vi "Main.vi"(8 "error in":errorcluster, 10 "User Events":T1, 11 "Message Queues in":T2) -> (0 "error out":errorcluster)   [LabVIEW 2026, in "UI.lvlib"]
doc: "This template is for the Queued Message Handler design pattern.\n\nThe Event Handling Loop generates messages based on user interface actions.\n\nThe Message Handling Loop processes messages generated by the Event Handling Loop, or by other messages. The messages are string values, so new messages can be added easily to the Message Cases case structure in the Message Handling Loop. Each message cluster can also provide an optional value for Message Data, which is a variant that can be converted to whatever message-specific data is required."
uses:
  UI.lvlib
  support/Message Queue/All Message Queues.ctl
  support/Message Queue/Message Cluster.ctl
  support/User Event - Stop/User Events.ctl
  Type Definitions/Data.ctl
  63137d18-bf8a-4e88-9200-6af118f85cfe.vi
  1e39ca58-9476-46a2-b025-c1705f3df17d.vi
  996e5f3e-9492-4e2b-97a9-5cb558c20b1f.vi
  73755cc0-1500-4328-8249-424498ba1049.vi
  5d810f25-301b-4729-8d99-398627275c85.vi
  4f3ed8a2-4889-49b4-8636-eb87dbb66537.vi
  c1dd759d-c855-4646-8354-c3344e12efab.vi
  4da0cbbb-3ae4-43c8-84ea-24bb95110d96.vi
  72e6443c-2ce6-4ed8-b611-5763f8d8c9de.vi
  63137d18-bf8a-4e88-9200-6af118f85cfe.vi/904feb24-0ee5-4d46-a973-81b984403c80.vi
  1e39ca58-9476-46a2-b025-c1705f3df17d.vi/904feb24-0ee5-4d46-a973-81b984403c80.vi
  996e5f3e-9492-4e2b-97a9-5cb558c20b1f.vi/904feb24-0ee5-4d46-a973-81b984403c80.vi
  73755cc0-1500-4328-8249-424498ba1049.vi/904feb24-0ee5-4d46-a973-81b984403c80.vi
  5d810f25-301b-4729-8d99-398627275c85.vi/904feb24-0ee5-4d46-a973-81b984403c80.vi
  4f3ed8a2-4889-49b4-8636-eb87dbb66537.vi/904feb24-0ee5-4d46-a973-81b984403c80.vi
  c1dd759d-c855-4646-8354-c3344e12efab.vi/904feb24-0ee5-4d46-a973-81b984403c80.vi
  4da0cbbb-3ae4-43c8-84ea-24bb95110d96.vi/904feb24-0ee5-4d46-a973-81b984403c80.vi
  72e6443c-2ce6-4ed8-b611-5763f8d8c9de.vi/904feb24-0ee5-4d46-a973-81b984403c80.vi
  support/Message Queue/Enqueue Message (Single).vi
  <vilib>/Utility/error.llb/Error Cluster From Error Code.vi
  <vilib>/ErrorRing/Error Ring.xnode
  support/Message Queue/Message Queue.lvlib
  support/User Event - Stop/User Event - Stop.lvlib
panel:
  out "Display <Replace Me>":string
  in  "Do Something Else <Replace Me>":bool
  in  "Do Something <Replace Me>":bool
  in  "Exit":bool
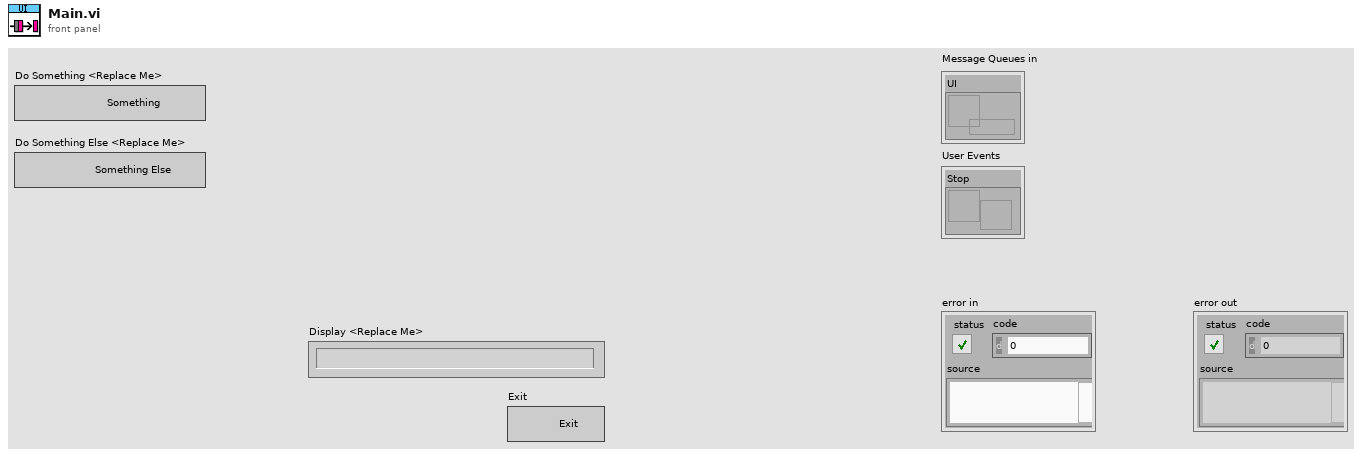
[diagram p1: front panel]
types:
  T1 = typedef "User Event - Stop.lvlib/User Events.ctl" = cluster{"Stop":refnum<user-event>}
  T2 = typedef "Message Queue.lvlib/All Message Queues.ctl" = cluster{"UI":refnum<queue>}
  T3 = enum32{"Invalid", "Standard", "Closed", "Hidden", "Minimized", "Maximized"}
  T4 = typedef "UI.lvlib/Data.ctl" = cluster{"Boolean <Replace Me>":bool, "String <Replace Me>":string, "Numeric <Replace Me>":dbl, "Do Something Ref":refnum<vi>, "Do Something Else Ref":refnum<vi>, "Exit Button Ref":refnum<vi>, "Display Ref":refnum<vi>}
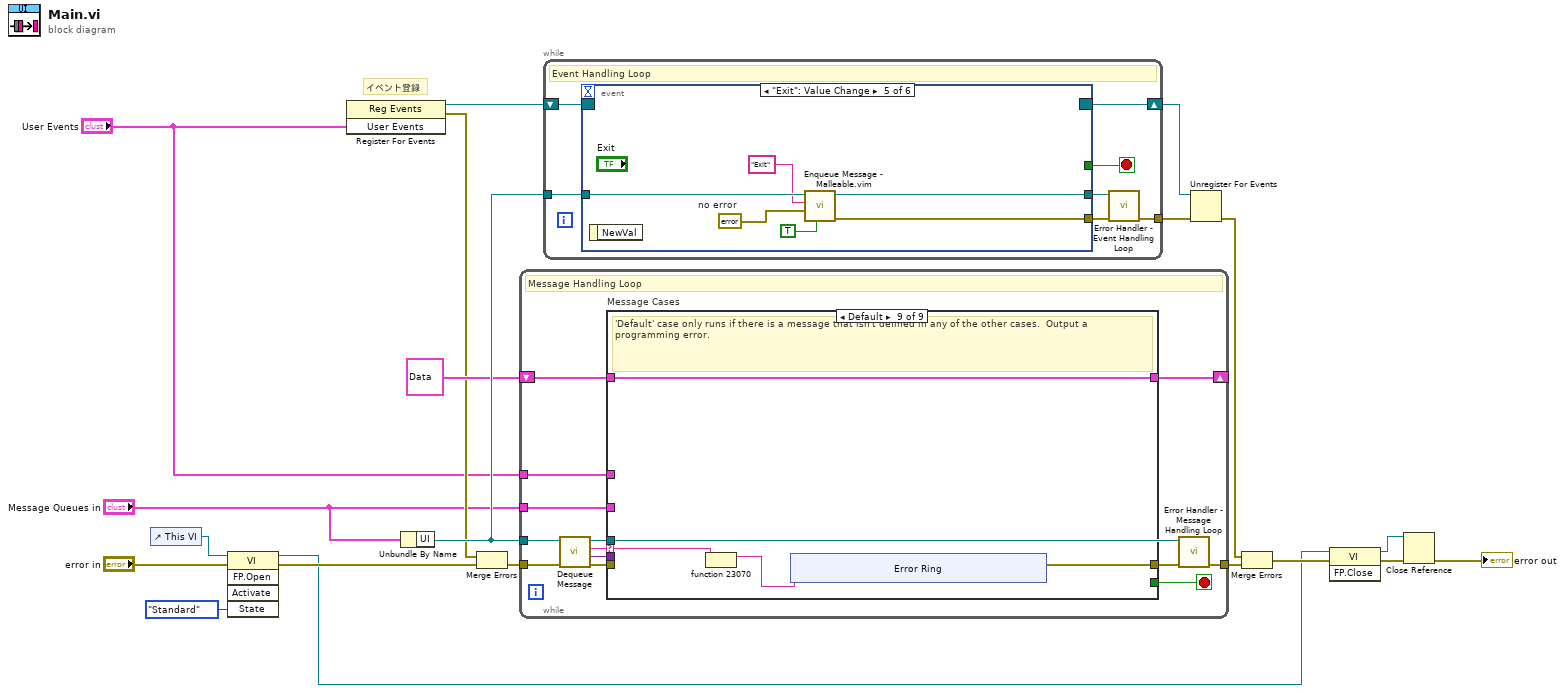
[diagram p0: block diagram]
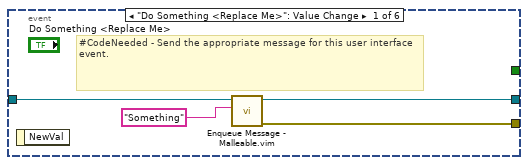
[diagram p2: hidden frame]
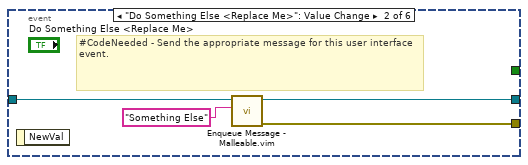
[diagram p3: hidden frame]
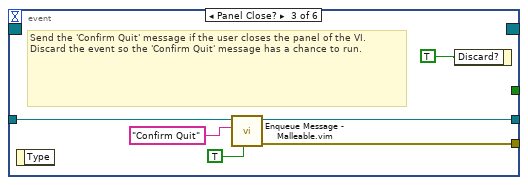
[diagram p4: hidden frame]
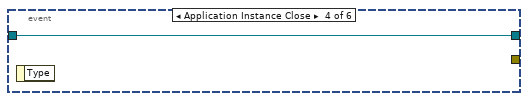
[diagram p5: hidden frame]
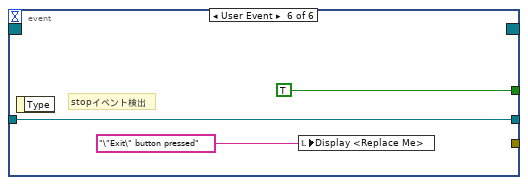
[diagram p6: hidden frame]
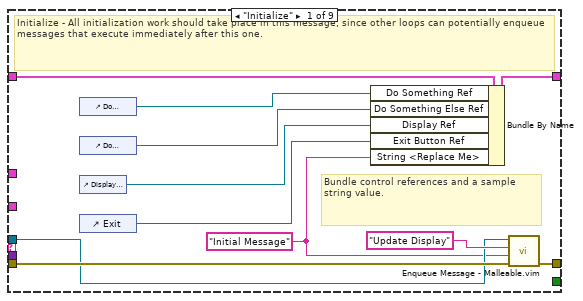
[diagram p7: hidden frame]
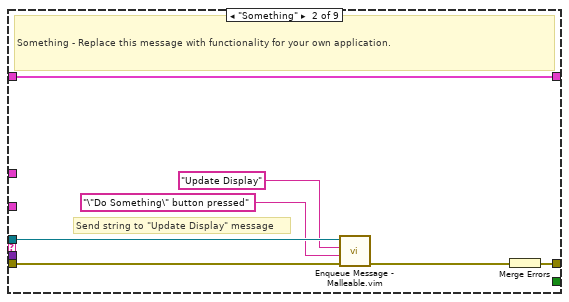
[diagram p8: hidden frame]
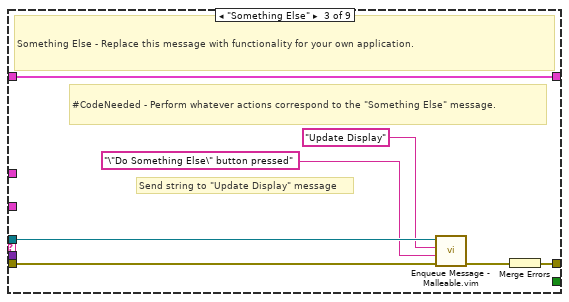
[diagram p9: hidden frame]
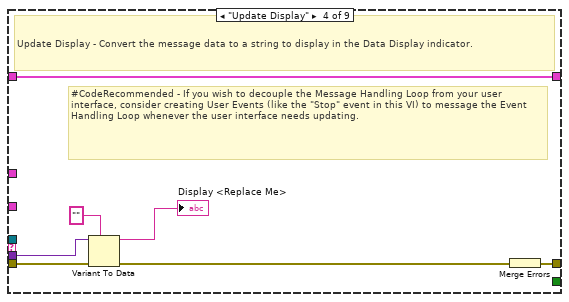
[diagram p10: hidden frame]
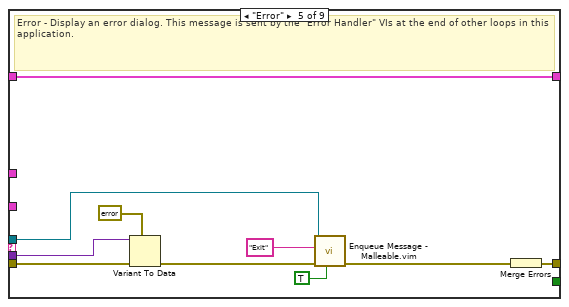
[diagram p11: hidden frame]
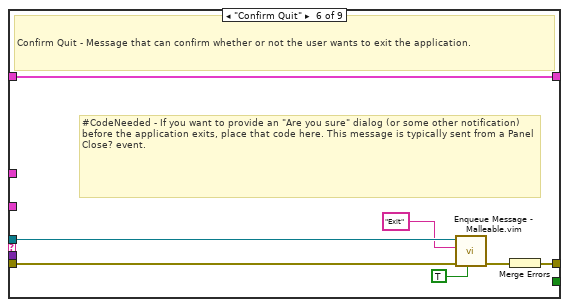
[diagram p12: hidden frame]
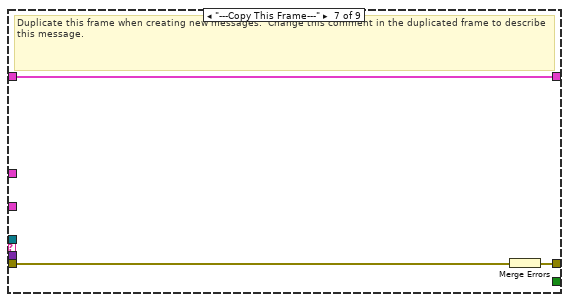
[diagram p13: hidden frame]
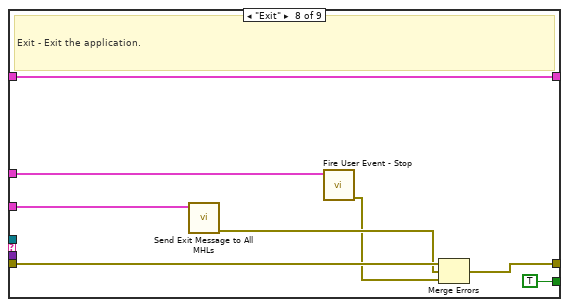
[diagram p14: hidden frame]
diagram:
  # "イベント登録"
  n1 = control-ref of="This VI"() -> (w6:refnum<vi>)
  n2 = invoke class="VI" method="FP.Open"(reference=w6, error in="error in", "State"=T3."Standard") -> (reference out=w4:refnum<vi>, error out=w7:errorcluster)  [unwired: 2 in, 3 out]
  n3 = register-events("User Events") -> (reference out=w14:refnum<event-registration>, error out=w12:errorcluster)  [unwired: 2 in]
  n4 = Unbundle By Name("Message Queues in") -> ("UI"=w19:refnum<queue>)
  n5 = Merge Errors(w12, w7) -> (w13:errorcluster)
  n6 = while {
    tunnel: w19 -> [w25]
    shift-right: [w32] -> _
    shift-left: T4 {"Boolean <Replace Me>"=FALSE, "String <Replace Me>"="", "Numeric <Replace Me>"=0.0, "Do Something Ref"=refnum, "Do Something Else Ref"=refnum, "Exit Button Ref"=refnum, "Display Ref"=refnum} ("Data Cluster") -> [w33]
    tunnel: "User Events" -> [w30]
    tunnel: w13 -> [w29]
    tunnel: [w23] -> w20
    tunnel: "Message Queues in" -> [w21]
    stop <- w31 stop-if-true
    # "Message Handling Loop"
    n7 = call "Dequeue Message.vi"("error in (no error)"=w29, "Message Queue"=w25) -> ("error out"=w28:errorcluster, "Message Data"=w26:variant, "Message"=w27:string, "dup Message Queue"=w24:refnum<queue>)  [unwired: 6 in]
    n8 = case "Message Cases" shown="Default" w27 {
      selector: w27 -> [_ _ _ _ _ _ _ _ w95]
      tunnel: w24 -> [w36 w48 w54 _ w69 w78 _ _ _]
      tunnel: w28 -> [w43 w49 w56 w63 w75 w82 w85 w88 _]
      tunnel: [w44 w50 w57 w64 w71 w80 w83 w91 w96] -> w22
      tunnel: w33 -> [w42 w51 w58 w65 w74 w81 w84 w93 w97]
      tunnel: [w41 w51 w58 w65 w74 w81 w84 w93 w97] -> w32
      tunnel: [_ _ _ _ _ _ _ TRUE _] -> w31
      tunnel: w26 -> [_ _ _ w62 w73 _ _ _ _]
      tunnel: w30 -> [_ _ _ _ _ _ _ w90 _]
      tunnel: w21 -> [_ _ _ _ _ _ _ w89 _]
      frame "Initialize" {
        w35 = "Initial Message" ("Initial Message")
        # "Bundle control references and a sample string value."
        # "Initialize - All initialization work should take place in this message, since other loops can potentially enqueue messages that execute immediately after this one."
        n9 = control-ref of="Do Something <Replace Me>"() -> (w40:refnum<vi>)
        n10 = control-ref of="Do Something Else <Replace Me>"() -> (w39:refnum<vi>)
        n11 = control-ref of="Display <Replace Me>"() -> (w34:refnum<vi>)
        n12 = control-ref of="Exit"() -> (w38:refnum<vi>)
        n13 = Bundle By Name(cluster=w42, "Do Something Ref"=w40, "Do Something Else Ref"=w39, "Display Ref"=w34, "Exit Button Ref"=w38, "String <Replace Me>"=w35) -> (w41:T4)
        n14 = call "Enqueue Message - Malleable.vim"("error in (no error)"=w43, "Message Data"=w35, "Message"="Update Display", "Message Queue"=w36) -> ("error out"=w44:errorcluster)  [unwired: 6 in, 1 out]
      }
      frame "Something" {
        # "Send string to \"Update Display\" message"
        # "Something - Replace this message with functionality for your own application."
        n15 = call "Enqueue Message - Malleable.vim"("error in (no error)"=w49, "Message Data"="\"Do Something\" button pressed" ("\"Do Something\" button pressed"), "Message"="Update Display", "Message Queue"=w48) -> ("error out"=w45:errorcluster)  [unwired: 6 in, 1 out]
        n16 = Merge Errors(w45) -> (w50:errorcluster)
      }
      frame "Something Else" {
        # "Send string to \"Update Display\" message"
        # "#CodeNeeded - Perform whatever actions correspond to the \"Something Else\" message."
        # "Something Else - Replace this message with functionality for your own application."
        n17 = call "Enqueue Message - Malleable.vim"("error in (no error)"=w56, "Message Data"="\"Do Something Else\" button pressed" ("\"Do Something Else\" button pressed"), "Message"="Update Display", "Message Queue"=w54) -> ("error out"=w55:errorcluster)  [unwired: 6 in, 1 out]
        n18 = Merge Errors(w55) -> (w57:errorcluster)
      }
      frame "Update Display" {
        # "#CodeRecommended - If you wish to decouple the Message Handling Loop from your user interface, consider creating User Events (like the \"Stop\" event in this VI) to message the Event Handling Loop whenever the user interface needs updating."
        # "Update Display - Convert the message data to a string to display in the Data Display indicator."
        n19 = Variant To Data(error in=w63, type="" ("data"), Variant=w62) -> (data=→"Display <Replace Me>":string, error out=w61:errorcluster)
        n20 = Merge Errors(w61) -> (w64:errorcluster)
      }
      frame "Error" {
        # "Error - Display an error dialog. This message is sent by the \"Error Handler\" VIs at the end of other loops in this application."
        n21 = Variant To Data(error in=w75, type=errorcluster {"status"=FALSE, "code"=0, "source"=""} ("error constant"), Variant=w73) -> (error out=w68:errorcluster)  [unwired: 1 out]
        n22 = call "Enqueue Message - Malleable.vim"("Priority Message? (F)"=TRUE, "error in (no error)"=w68, "Message"="Exit", "Message Queue"=w69) -> ("error out"=w67:errorcluster)  [unwired: 6 in, 1 out]
        n23 = Merge Errors(w67) -> (w71:errorcluster)
      }
      frame "Confirm Quit" {
        # "#CodeNeeded - If you want to provide an \"Are you sure\" dialog (or some other notification) before the application exits, place that code here. This message is typically sent from a Panel Close? event."
        # "Confirm Quit - Message that can confirm whether or not the user wants to exit the application."
        n24 = call "Enqueue Message - Malleable.vim"("Priority Message? (F)"=TRUE, "error in (no error)"=w82, "Message"="Exit", "Message Queue"=w78) -> ("error out"=w79:errorcluster)  [unwired: 6 in, 1 out]
        n25 = Merge Errors(w79) -> (w80:errorcluster)
      }
      frame "---Copy This Frame---" {
        # "Duplicate this frame when creating new messages.  Change this comment in the duplicated frame to describe this message."
        n26 = Merge Errors(w85) -> (w83:errorcluster)
      }
      frame "Exit" {
        # "Exit - Exit the application."
        n27 = call "Send Exit Message to All MHLs.vi"("Message Queues"=w89) -> ("error out"=w87:errorcluster)  [unwired: 10 in]
        n28 = call "Fire User Event - Stop.vi"("User Events"=w90) -> ("error out"=w86:errorcluster)  [unwired: 10 in]
        n29 = Merge Errors(w88, w87, w86) -> (w91:errorcluster)
      }
      frame Default {
        # "'Default' case only runs if there is a message that isn't defined in any of the other cases.  Output a programming error."
        n30 = fn#23070(3:w95) -> (0:w94:string)  [unwired: 1 in, 1 out]
        n31 = xnode "Error Ring"("parameter 0"=w94) -> ("error out"=w96:errorcluster)
      }
    }
    n32 = call "Error Handler - Message Handling Loop.vi"("error in (no error)"=w22, "Message Queue"=w24) -> ("dup error in"=w23:errorcluster)  [unwired: 8 in, 1 out]
  }
  n33 = while {
    tunnel: w19 -> [w111]
    shift-right: [w105] -> w17
    shift-left: w14 -> [w106]
    tunnel: [w107] -> w15
    stop <- w109 stop-if-true
    # "Event Handling Loop"
    n34 = event shown="[4] \"Exit\": Value Change" {
      selector: w106 -> [_ _ _ _ _ _]
      dyn-events: [_ _ _ _ _ _] -> w105
      timeout: _ -> [_ _ _ _ _ _]
      tunnel: [_ _ _ _ _ TRUE ("Discard?")] -> w109
      tunnel: w111 -> [w115 w119 w124 w126 w132 w135]
      tunnel: [w112 w116 w123 _ w131 _] -> w110
      tunnel: [w114 w118 w122 w126 w130 w135] -> w108
      event "Do Something <Replace Me>": Value Change {
        # "#CodeNeeded - Send the appropriate message for this user interface event."
        n35 = event-data() -> ()  [unwired: 1 in, 1 out]
        n36 = call "Enqueue Message - Malleable.vim"("Message"="Something", "Message Queue"=w115) -> ("error out"=w112:errorcluster, "dup Message Queue"=w114:refnum<queue>)  [unwired: 8 in]
      }
      event "Do Something Else <Replace Me>": Value Change {
        # "#CodeNeeded - Send the appropriate message for this user interface event."
        n37 = event-data() -> ()  [unwired: 1 in, 1 out]
        n38 = call "Enqueue Message - Malleable.vim"("Message"="Something Else", "Message Queue"=w119) -> ("error out"=w116:errorcluster, "dup Message Queue"=w118:refnum<queue>)  [unwired: 8 in]
      }
      event Panel Close? {
        # "Send the 'Confirm Quit' message if the user closes the panel of the VI. Discard the event so the 'Confirm Quit' message has a chance to run."
        n39 = event-data() -> ()  [unwired: 1 in, 1 out]
        n40 = call "Enqueue Message - Malleable.vim"("Priority Message? (F)"=TRUE, "Message"="Confirm Quit", "Message Queue"=w124) -> ("error out"=w123:errorcluster, "dup Message Queue"=w122:refnum<queue>)  [unwired: 7 in]
        n41 = event-data("Discard?"=TRUE) -> ()  [unwired: 1 in, 1 out]
      }
      event Application Instance Close {
        n42 = event-data() -> ()  [unwired: 1 in, 1 out]
      }
      event "Exit": Value Change {
        w127 = errorcluster {"status"=FALSE, "code"=0, "source"=""}  # no error
        n43 = event-data() -> ()  [unwired: 1 in, 1 out]
        n44 = call "Enqueue Message - Malleable.vim"("Priority Message? (F)"=TRUE, "Message Data"=w127, "Message"="Exit", "Message Queue"=w132) -> ("error out"=w131:errorcluster, "dup Message Queue"=w130:refnum<queue>)  [unwired: 6 in]
      }
      event User Event {
        # "stopイベント検出"
        n45 = event-data() -> ()  [unwired: 1 in, 1 out]
        n46 = local write "Display <Replace Me>"("\"Exit\" button pressed" ("VI Stopped")) -> ()
      }
    }
    n47 = call "Error Handler - Event Handling Loop.vi"("error in (no error)"=w110, "Message Queue"=w108) -> ("dup error in"=w107:errorcluster)  [unwired: 8 in, 1 out]
  }
  n48 = Unregister For Events(event registration refnum=w17, error in=w15) -> (error out=w18:errorcluster)
  n49 = Merge Errors(w18, w20) -> (w5:errorcluster)
  n50 = invoke class="VI" method="FP.Close"(reference=w4, error in=w5) -> (reference out=w2:refnum<vi>, error out=w3:errorcluster)  [unwired: 1 in, 1 out]
  n51 = Close Reference(reference=w2, error in (no error)=w3) -> (error out=→"error out":errorcluster)
